vi "Report Event.vi"(7 "Level (Info)":T1=enum."Info", 8 "error in (no error)":errorcluster, 9 "Message":string, 10 "Context":string, 11 "VolatusAPI in":refnum<class "VolatusAPI.lvclass">) -> (0 "error out":errorcluster, 3 "VolatusAPI out":refnum<class "VolatusAPI.lvclass">)   [LabVIEW 2020, in "Volatus.lvlib" / "VolatusAPI.lvclass"]
uses:
  VolatusAPI.lvclass
  Event Level.ctl
  Event.ctl
  VolatusAPI.lvclass/VolatusAPI.ctl
  MessageQ/MessageQ.lvclass/MessageQ.ctl
  Volatus.lvlib
  MessageQ/MessageQ.lvclass
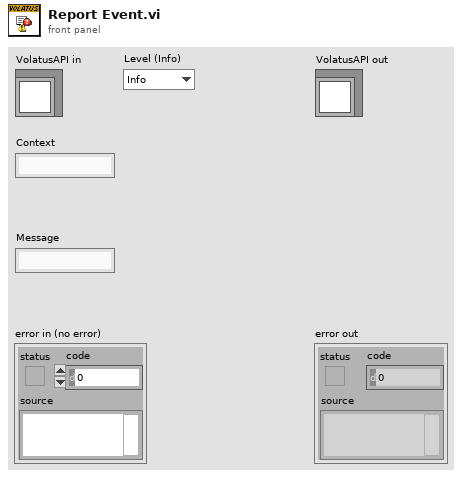
[diagram p1: front panel]
types:
  T1 = typedef "Volatus.lvlib/Event Level.ctl" = enum16{"Debug", "Info", "Warning", "Error"}
  T2 = typedef "Volatus.lvlib/Event.ctl" = cluster{"Time Stamp":timestamp, "Event Level":T1, "Context":string, "Message":string, "Error":errorcluster, "Node":string}
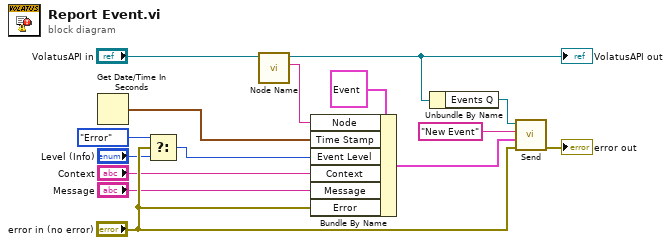
[diagram p0: block diagram]
diagram:
  n1 = Get Date/Time In Seconds() -> (seconds since 1Jan1904=w7:timestamp)
  n2 = Select(t=Event_Level."Error", s="error in (no error)", f="Level (Info)") -> (s? t:f=w4:T1)
  n3 = call "Node Name.vi"("VolatusAPI in"="VolatusAPI in") -> ("Node Name"=w1:string, "VolatusAPI out"=w2:refnum<class "VolatusAPI.lvclass">)  [unwired: 8 in, 1 out]
  "VolatusAPI out" <- w2
  n4 = Bundle By Name(cluster=T2 {"Time Stamp"=timestamp(0 s since 1904-01-01), "Event Level"=enum."Info", "Context"="", "Message"="", "Error"={"status"=FALSE, "code"=0, "source"=""}, "Node"=""} ("Event"), "Node"=w1, "Time Stamp"=w7, "Event Level"=w4, "Context"="Context", "Message"="Message", "Error"="error in (no error)") -> (w9:T2)
  n5 = Unbundle By Name(w2) -> ("Events Q"=w11:refnum<class "MessageQ.lvclass">)
  n6 = call "Send.vi"("error in (no error)"="error in (no error)", "Data"=w9, "ID"="New Event", "MessageQ in"=w11) -> ("error out"=→"error out":errorcluster)  [unwired: 6 in, 1 out]
